vi "global.vi"() -> ()   [LabVIEW 2025]
uses:
  System.Windows.Forms
panel:
  in  "ModbusConfig":T1(array[cluster])=[{"Name"="最大电流", "Type"="BOL", "DefVal"="T"}, {"Name"="平均电流", "Type"="BOL", "DefVal"="T"}, {"Name"="能量", "Type"="BOL", "DefVal"="T"}, {"Name"="打钉时间", "Type"="BOL", "DefVal"="T"}, {"Name"="单发打钉次数", "Type"="UINT", "DefVal"="10"}, {"Name"="触发值", "Type"="DBL", "DefVal"="8"}, {"Name"="平均电流上限", "Type"="DBL", "DefVal"="40"}, {"Name"="平均电流下限", "Type"="DBL", "DefVal"="0"}, {"Name"="最大电流上限", "Type"="DBL", "DefVal"="200"}, {"Name"="最大电流下限", "Type"="DBL", "DefVal"="0"}, {"Name"="能量上限", "Type"="DBL", "DefVal"="15"}, {"Name"="能量下限", "Type"="DBL", "DefVal"="0"}, {"Name"="时间上限", "Type"="DBL", "DefVal"="500"}, {"Name"="时间下限", "Type"="DBL", "DefVal"="0"}, {"Name"="连发打钉次数", "Type"="UINT", "DefVal"="0"}, {"Name"="停止值", "Type"="DBL", "DefVal"="1"}, {"Name"="倍数", "Type"="DBL", "DefVal"="1"}, {"Name"="最大补偿", "Type"="DBL", "DefVal"="0"}, {"Name"="平均补偿", "Type"="DBL", "DefVal"="0"}, {"Name"="能量补偿", "Type"="DBL", "DefVal"="0"}, {"Name"="时间补偿", "Type"="DBL", "DefVal"="0"}, {"Name"="检查数", "Type"="UINT", "DefVal"="20"}, {"Name"="CurrentType", "Type"="UINT", "DefVal"="0"}]
  out "ChangeDone":bool
  out "register parameter":u16[](array[numeric])
  in  "Modbus RTU Address":string
  in  "Low Volt alarm (0.01V)":string
  in  "High Volt alarm (0.01V)":string
  in  "Currrent Range":string(combo)
  out "HighAlarm":bool
  out "LowAlarm":bool
  out "Current(A)":dbl
  out "Voltage(V)":dbl
  out "Power(W)":dbl
  out "Energy(Wh)":dbl
  out "register data":u16[](array[numeric])
  out "RawDataPath":path
  out "Modbus":string
  in  "Para":T2
  in  "输入通道":tag="Dev2/ai0"
  in  "项目":refnum<vi>
  out "Start":bool
  out "AppPath":path
  in  "PassY":refnum<k24>
  in  "ConfigPara":T1(array[cluster])=[{"Name"="最大电流", "Type"="BOL", "DefVal"="T"}, {"Name"="平均电流", "Type"="BOL", "DefVal"="T"}, {"Name"="能量", "Type"="BOL", "DefVal"="T"}, {"Name"="打钉时间", "Type"="BOL", "DefVal"="T"}, {"Name"="单发打钉次数", "Type"="UINT", "DefVal"="10"}, {"Name"="触发值", "Type"="DBL", "DefVal"="8"}, {"Name"="平均电流上限", "Type"="DBL", "DefVal"="40"}, {"Name"="平均电流下限", "Type"="DBL", "DefVal"="0"}, {"Name"="最大电流上限", "Type"="DBL", "DefVal"="200"}, {"Name"="最大电流下限", "Type"="DBL", "DefVal"="0"}, {"Name"="能量上限", "Type"="DBL", "DefVal"="15"}, {"Name"="能量下限", "Type"="DBL", "DefVal"="0"}, {"Name"="时间上限", "Type"="DBL", "DefVal"="500"}, {"Name"="时间下限", "Type"="DBL", "DefVal"="0"}, {"Name"="连发打钉次数", "Type"="UINT", "DefVal"="0"}, {"Name"="停止值", "Type"="DBL", "DefVal"="1"}, {"Name"="倍数", "Type"="DBL", "DefVal"="1"}, {"Name"="最大补偿", "Type"="DBL", "DefVal"="0"}, {"Name"="平均补偿", "Type"="DBL", "DefVal"="0"}, {"Name"="能量补偿", "Type"="DBL", "DefVal"="0"}, {"Name"="时间补偿", "Type"="DBL", "DefVal"="0"}, {"Name"="检查数", "Type"="UINT", "DefVal"="20"}, {"Name"="CurrentType", "Type"="UINT", "DefVal"="0"}]
  out "language":string
  out "PLC":string
  in  "Pass":refnum<k24>
  in  "Fail":refnum<k24>
  in  "Text":refnum<k24>
  out "DataPath":path
  out "ReportPath":path
  out "ConfigPath":path
  out "Stop?":bool
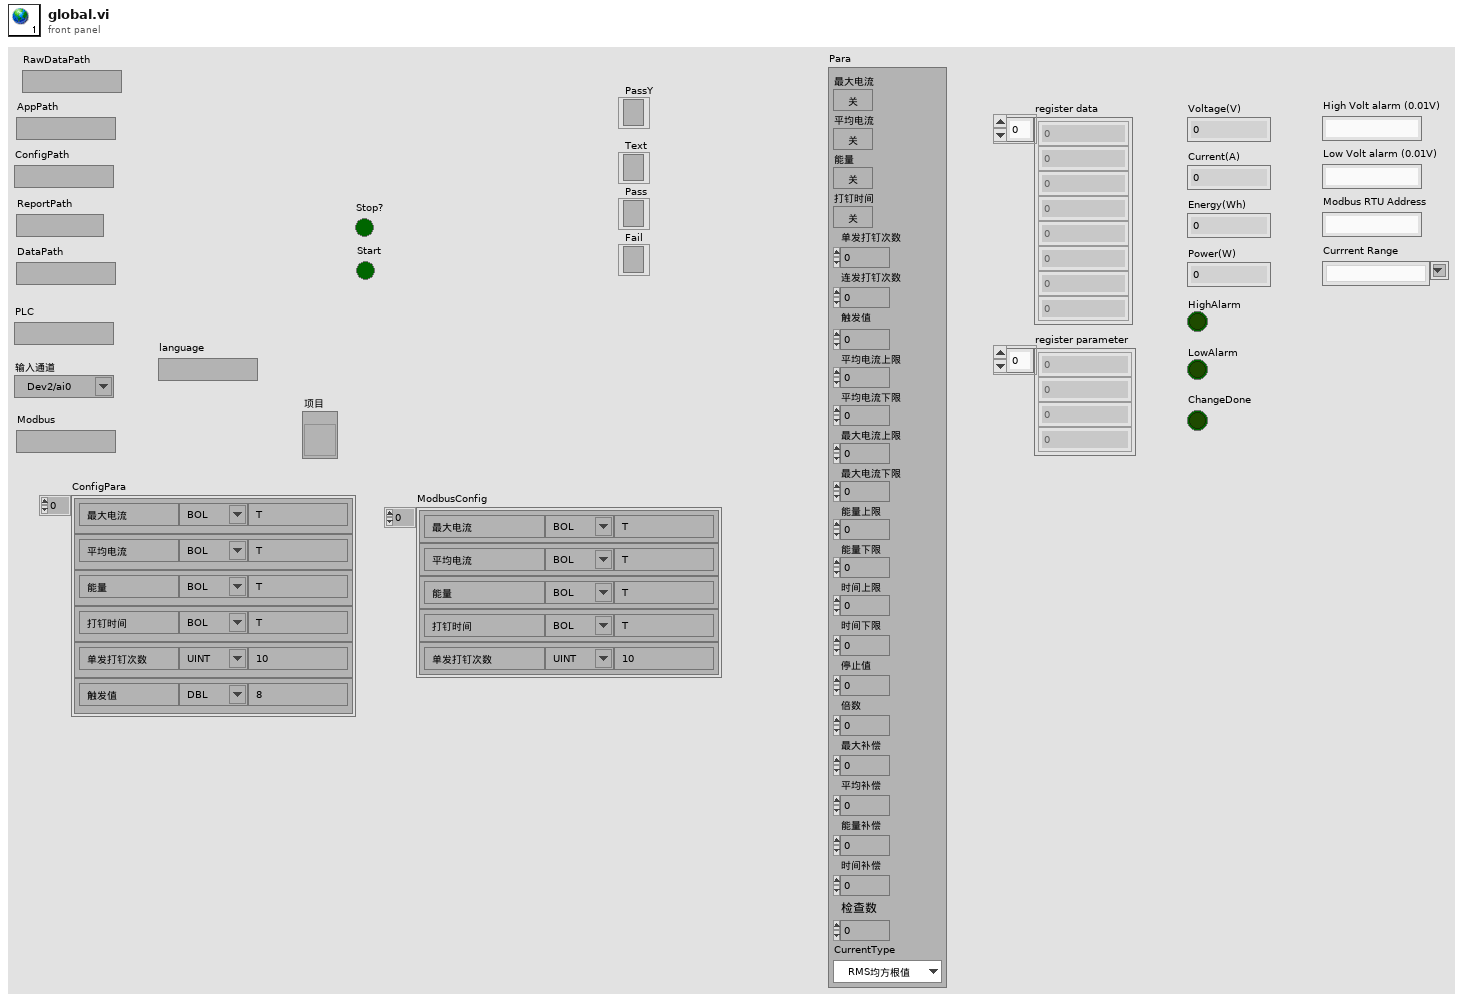
[diagram p1: front panel]
types:
  T1 = cluster{"Name":string, "Type":string, "DefVal":string}[]
  T2 = cluster{"最大电流":bool, "平均电流":bool, "能量":bool, "打钉时间":bool, "单发打钉次数":u32, "连发打钉次数":u32, "触发值":dbl, "平均电流上限":dbl, "平均电流下限":dbl, "最大电流上限":dbl, "最大电流下限":dbl, "能量上限":dbl, "能量下限":dbl, "时间上限":dbl, "时间下限":dbl, "停止值":dbl, "倍数":dbl, "最大补偿":dbl, "平均补偿":dbl, "能量补偿":dbl, "时间补偿":dbl, "检查数":u32, "CurrentType":enum16{"RMS均方根值", "AVG平均值"}}
diagram:
